vi "R_procotol.vi"(8 "error in (no error)":errorcluster caption="错误输入（无错误）", 11 "Procotol_class 输入":refnum<class "Procotol_class.lvclass">) -> (0 "error out":errorcluster caption="错误输出", 3 "Procotol_class 输出":refnum<class "Procotol_class.lvclass">)   [LabVIEW 2025, in "Procotol_class.lvclass"]
uses:
  Procotol_class.lvclass
  <vilib>/Utility/NIReport.llb/Report Type.ctl
  Procotol_class.lvclass/Procotol_class.ctl
  <vilib>/addons/_office/excel.llb/Excel Get Data ([str]).vi
  <vilib>/Utility/NIReport.llb/NI_report.lvclass
  <vilib>/Utility/NIReport.llb/NI_ReportGenerationCore.lvlib
  <vilib>/Utility/NIReport.llb/Excel/NI_Excel.lvclass
  <vilib>/addons/_office/NI_ReportGenerationToolkit.lvlib
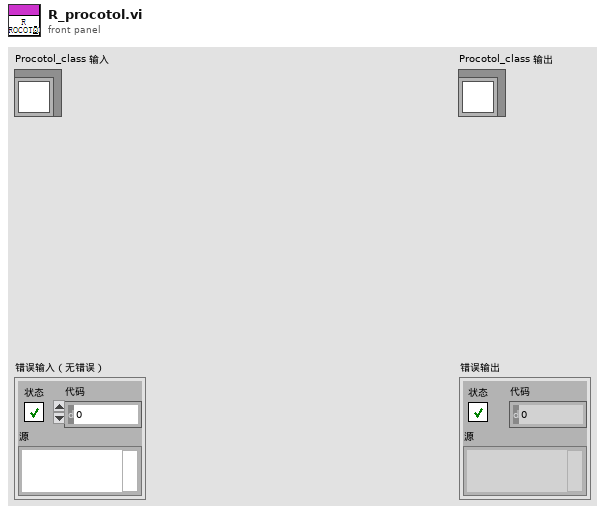
[diagram p1: front panel]
types:
  T1 = typedef "NI_ReportGenerationCore.lvlib/Report Type.ctl" = enum16{"HTML", "Word", "Excel"}
  T2 = enum16{"maximized", "minimized", "normal", "no change"}
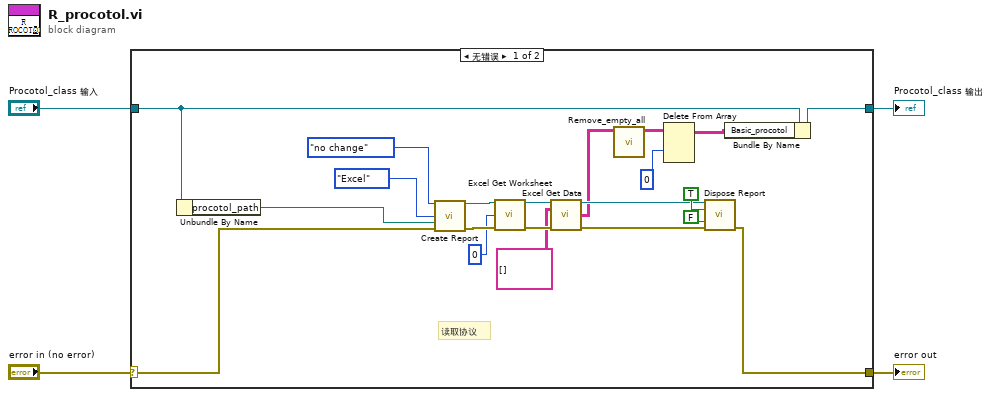
[diagram p0: block diagram]
diagram:
  n1 = case shown="无错误" "error in (no error)" {
    selector: "error in (no error)" -> [w21 w27]
    tunnel: [w9 w27] -> w3
    tunnel: [w20 w26] -> w1
    tunnel: "Procotol_class 输入" -> [w23 w26]
    frame No Error {
      # "读取协议"
      n2 = Unbundle By Name(w23) -> ("procotol_path"=w22:path)
      n3 = call <vilib>:"Create Report.vi"("window state (normal)"=T2."no change", "report type"=Report_Type."Excel", "template (empty)"=w22, "error in (no error)"=w21) -> ("report out"=w19:refnum<class "NI_report.lvclass">, "error out"=w18:errorcluster)  [unwired: 10 in]
      n4 = call <vilib>:"Excel Get Worksheet.vi"("report in"=w19, "worksheet index (0)"=0, "error in (no error)"=w18) -> ("report out"=w16:refnum<class "NI_report.lvclass">, "error out"=w15:errorcluster)  [unwired: 11 in]
      n5 = call-poly <vilib>:"Excel Get Data.vi"("report in"=w16, "data type"=string[][] [], "error in (no error)"=w15) -> ("report out"=w10:refnum<class "NI_report.lvclass">, "data"=w8:string[][], "error out"=w11:errorcluster)  [unwired: 10 in]
      n6 = call "Remove_empty_all.vi"("ARR_in"=w8) -> ("ARR_out"=w7:string[][])  [unwired: 10 in]
      n7 = Delete From Array(array=w7, index (row)=0 ("索引 (行)")) -> (array with subset deleted=w6:string[][])  [unwired: 2 in, 1 out]
      n8 = call-dynamic "Dispose Report.vi"("report in"=w10, "wait until printing completed? (T)"=TRUE, "save changes? (F)"=FALSE, "error in (no error)"=w11) -> ("error out"=w9:errorcluster)  [unwired: 11 in]
      n9 = Bundle By Name(cluster=w23, "Basic_procotol"=w6) -> (w20:refnum<class "Procotol_class.lvclass">)
    }
    frame Error {
    }
  }
  "error out" <- w3
  "Procotol_class 输出" <- w1
